vi "getTitleImage.vi"(3 "error in (no error)":errorcluster caption="错误输入（无错误）", 4 "story":T1) -> (0 "title":string, 1 "error out":errorcluster caption="错误输出", 2 "图片":picture)   [LabVIEW 2012]
panel:
  out "响应体":string
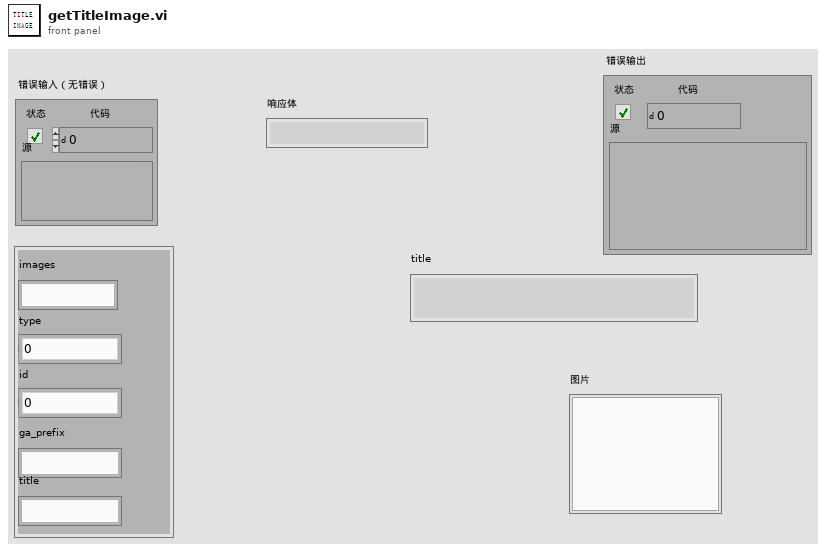
[diagram p1: front panel]
types:
  T1 = cluster{"images":string, "type":i32, "id":i64, "ga_prefix":string, "title":string}
  T2 = typedef "imagedata.ctl" = cluster{"image type":i32, "image depth":i32, "image":u8[], "mask":u8[], "colors":u32[], "Rectangle":cluster{"left":i16, "top":i16, "right":i16, "bottom":i16}}
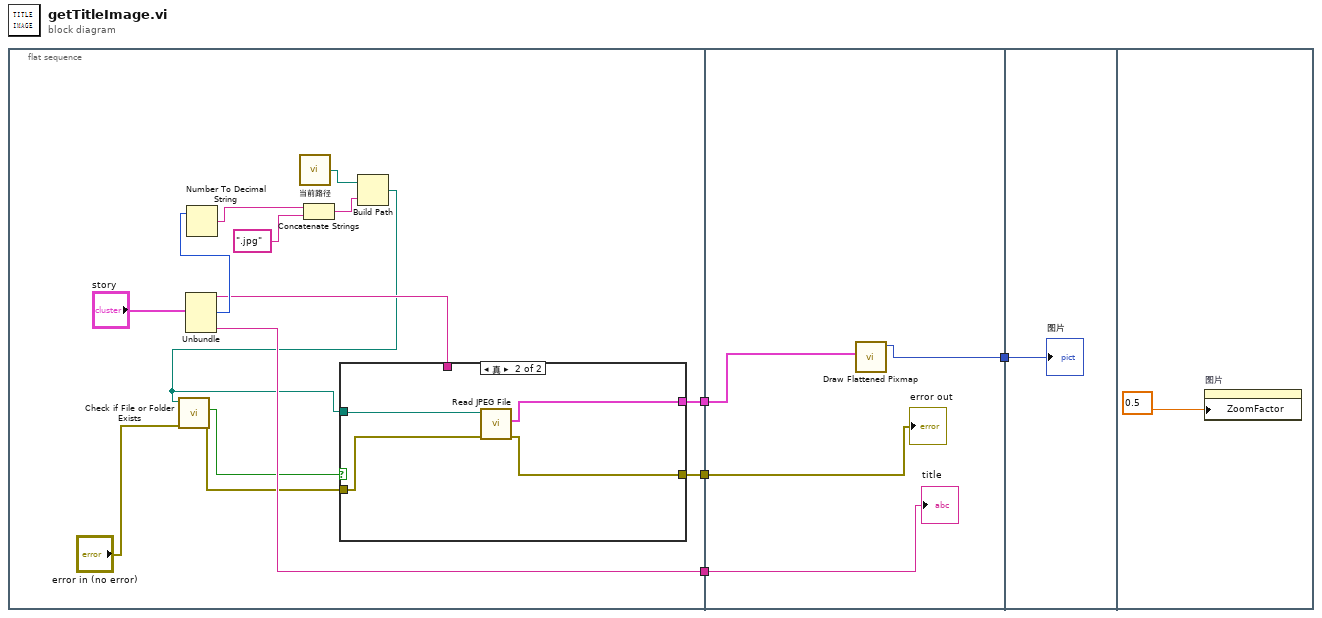
[diagram p0: block diagram]
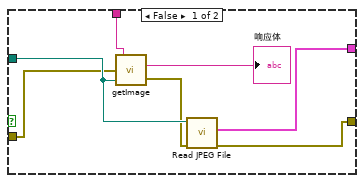
[diagram p2: hidden frame]
diagram:
  n1 = flat-sequence {
    tunnel: [w16] -> w3
    tunnel: [w15] -> w2
    tunnel: [w13] -> w1
    tunnel: [w33] -> w4
    tunnel: w3 -> [w32]
    tunnel: w2 -> [w31]
    tunnel: w1 -> [w30]
    tunnel: w4 -> [w34]
    frame #0 {
      n2 = Unbundle("story") -> ("images"=w14:string, "id"=w17:i64, "title"=w13:string)  [unwired: 2 out]
      n3 = Number To Decimal String(number=w17) -> (decimal integer string=w6:string)  [unwired: 1 in]
      n4 = call "当前路径.vi"() -> ("路径"=w11:path)
      n5 = Concatenate Strings(w6, ".jpg") -> (w12:string)
      n6 = Build Path(base path=w11, name or relative path=w12) -> (appended path=w7:path)
      n7 = call <vilib>:"Check if File or Folder Exists.vi"("error in (no error)"="error in (no error)", "path"=w7) -> ("error out"=w8:errorcluster, "file or folder exists?"=w9:bool)  [unwired: 7 in, 1 out]
      n8 = case shown="真" w9 {
        tunnel: [w21 w27] -> w16
        tunnel: [w20 w26] -> w15
        tunnel: w7 -> [w23 w29]
        tunnel: w14 -> [w25 _]
        tunnel: w8 -> [w19 w28]
        frame False {
          n9 = call "getImage.vi"("路径"=w23, "error in (no error)"=w19, "URL"=w25) -> ("error out"=w22:errorcluster, "响应体"=→"响应体":string)
          n10 = call <vilib>:"Read JPEG File.vi"("error in (no error)"=w22, "path to JPEG file"=w23) -> ("error out"=w20:errorcluster, "image data"=w21:T2)  [unwired: 7 in, 1 out]
        }
        frame True {
          n11 = call <vilib>:"Read JPEG File.vi"("error in (no error)"=w28, "path to JPEG file"=w29) -> ("error out"=w26:errorcluster, "image data"=w27:T2)  [unwired: 7 in, 1 out]
        }
      }
    }
    frame #1 {
      n12 = call <vilib>:"Draw Flattened Pixmap.vi"("image data"=w32) -> ("new picture"=w33:picture)  [unwired: 8 in]
      "title" <- w30
      "error out" <- w31
    }
    frame #2 {
      "图片" <- w34
    }
    frame #3 {
      n13 = property on="图片" class="Pict"("ZoomFactor"=0.5) -> ()  [unwired: 2 in, 2 out]
    }
  }
